vi "close.vi"(8 "error in (no error)":errorcluster, 11 "Table in":refnum<class "Table.lvclass">) -> (0 "error out":errorcluster)   [LabVIEW 2020, in "toml_edit.lvlib" / "Table.lvclass"]
uses:
  Table.lvclass
  Table.lvclass/Table.ctl
  dragon_toml_64.dll
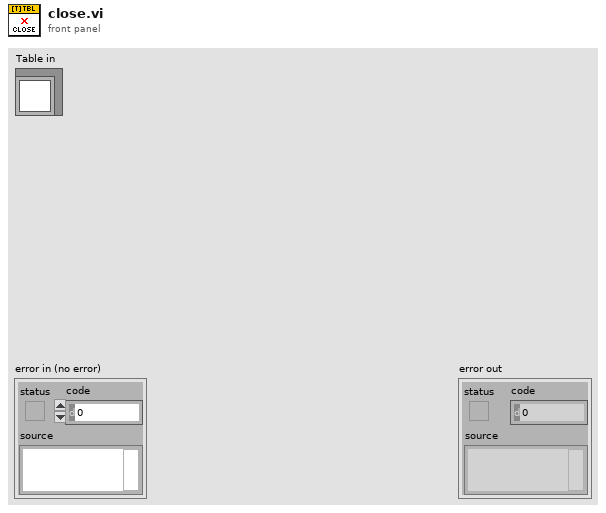
[diagram p1: front panel]
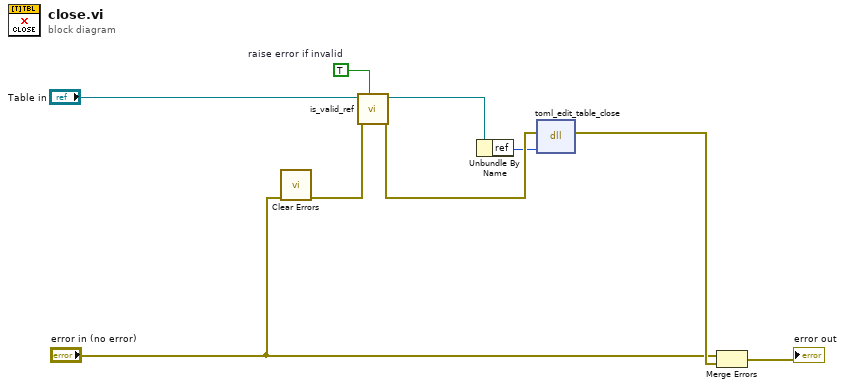
[diagram p0: block diagram]
diagram:
  w1 = TRUE  # raise error if invalid
  n1 = call <vilib>:"Clear Errors.vi"("error in (no error)"="error in (no error)") -> ("error out"=w4:errorcluster)  [unwired: 5 in, 1 out]
  n2 = call-dynamic "is_valid_ref.vi"("raise error if invalid? (False)"=w1, "error in (no error)"=w4, "Table in"="Table in") -> ("error out"=w3:errorcluster, "Table out"=w5:refnum<class "Table.lvclass">)  [unwired: 6 in, 1 out]
  n3 = Unbundle By Name(w5) -> ("ref"=w2:u64)
  n4 = dll-call lib="C:/projects/dragon-desktop/source/submodules/toml-edit-labview/lv_src/dragon_toml_*.dll" fn="toml_edit_table_close"(error in=w3, "table_ref"=w2) -> (error out=w9:errorcluster)  [unwired: 4 in, 1 out]
  n5 = Merge Errors("error in (no error)", w9) -> (→"error out":errorcluster)
